vi "Report_Export.vi"(8 "error in (no error)":errorcluster={"status"=FALSE, "code"=0, "source"="\"\""}, 10 "formatting template":string, 11 "Final result records":string) -> (0 "error out":errorcluster={"status"=FALSE, "code"=0, "source"="\"\""}, 2 "status ok":bool, 3 "CSV/HTML/PDF via separate approved converter":string)   [LabVIEW 2026]
doc: "INTENT: Produce operator-readable report. LOGIC: Summarize metadata, measurements, PASS/FAIL/INCOMPLETE and exception history."
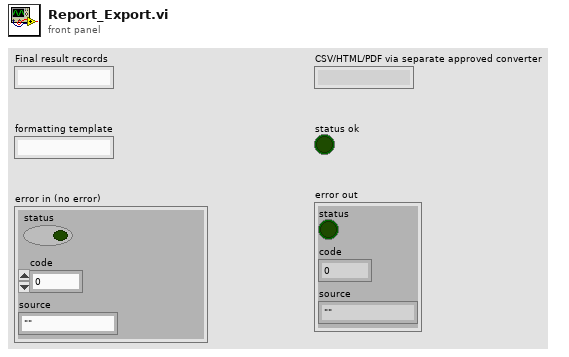
[diagram p1: front panel]
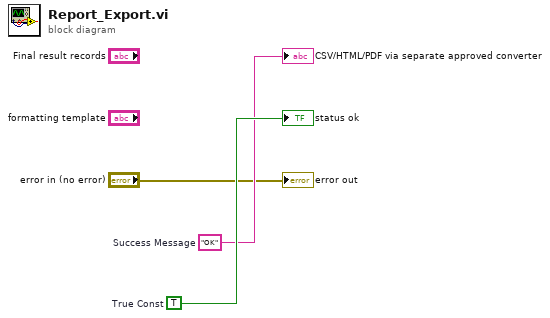
[diagram p0: block diagram]
diagram:
  w3 = TRUE  # True Const
  w2 = "OK"  # Success Message
  "CSV/HTML/PDF via separate approved converter" <- w2
  "status ok" <- w3
  "error out" <- "error in (no error)"
